vi "Enregistrer_fichier_profil EPC3000.vi"(2 "error in (no error) 2":errorcluster caption="entrée d'erreur (pas d'erreur)", 3 "Config + programmes":T1 {"Prog 10 en sortie"."?" format="%#.1f"; "Prog 9 en sortie"."?" format="%#.1f"; "Prog 8 en sortie"."?" format="%#.1f"; "Prog 7 en sortie"."?" format="%#.1f"; "Prog 6 en sortie"."?" format="%#.1f"; "Prog 5 en sortie"."?" format="%#.1f"; "config"."value" format="%#.1f"; "Prog 1 en sortie"."?" format="%#.1f"; "Prog 2 en sortie"."?" format="%#.1f"; "Prog 3 en sortie"."?" format="%#.1f"; "Prog 4 en sortie"."?" format="%#.1f"}, 4 "Chemin du fichier profil":path caption="chemin du fichier de configuration") -> (0 "error out 2":errorcluster caption="entrée d'erreur (pas d'erreur)", 1 "Chemin de fichier en sortie":path caption="Chemin du fichier en sortie")   [LabVIEW 2022 SP3]
uses:
  <vilib>/Utility/config.llb/Write Key (Double).vi
  <vilib>/Utility/config.llb/NI_LVConfig.lvlib
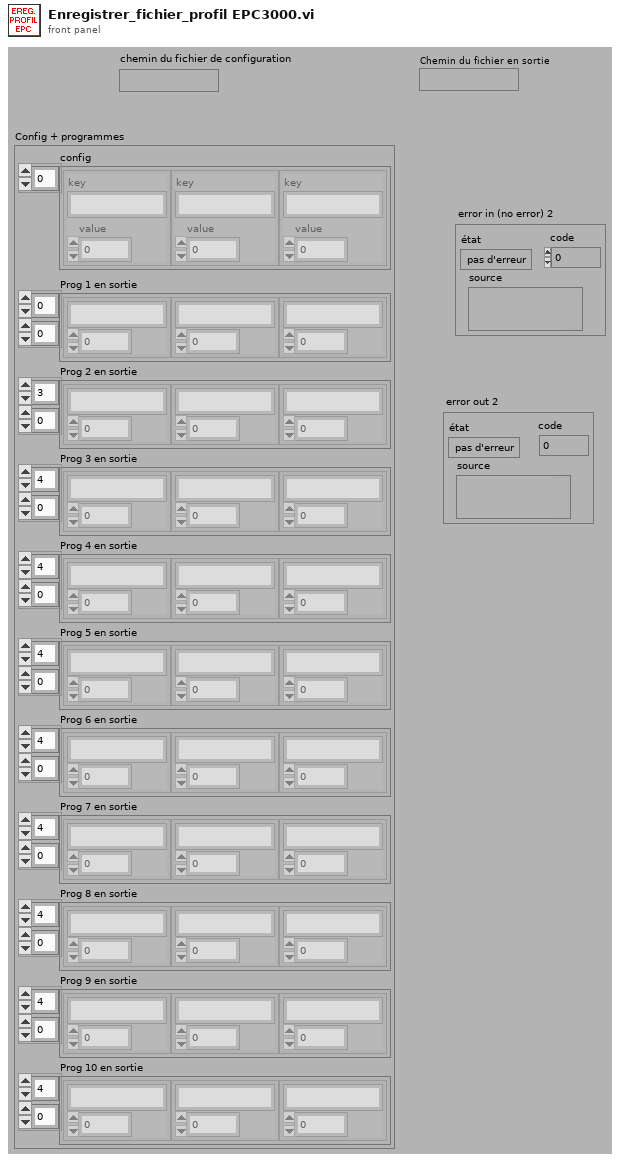
[diagram p1: front panel]
types:
  T1 = cluster{"config":cluster{"key":string, "value":dbl}[], "Prog 1 en sortie":cluster{string, dbl}[][], "Prog 2 en sortie":cluster{string, dbl}[][], "Prog 3 en sortie":cluster{string, dbl}[][], "Prog 4 en sortie":cluster{string, dbl}[][], "Prog 5 en sortie":cluster{string, dbl}[][], "Prog 6 en sortie":cluster{string, dbl}[][], "Prog 7 en sortie":cluster{string, dbl}[][], "Prog 8 en sortie":cluster{string, dbl}[][], "Prog 9 en sortie":cluster{string, dbl}[][], "Prog 10 en sortie":cluster{string, dbl}[][]}
  T2 = typedef "NI_LVConfig.lvlib/Config Data RefNum.ctl" = refnum<k1>
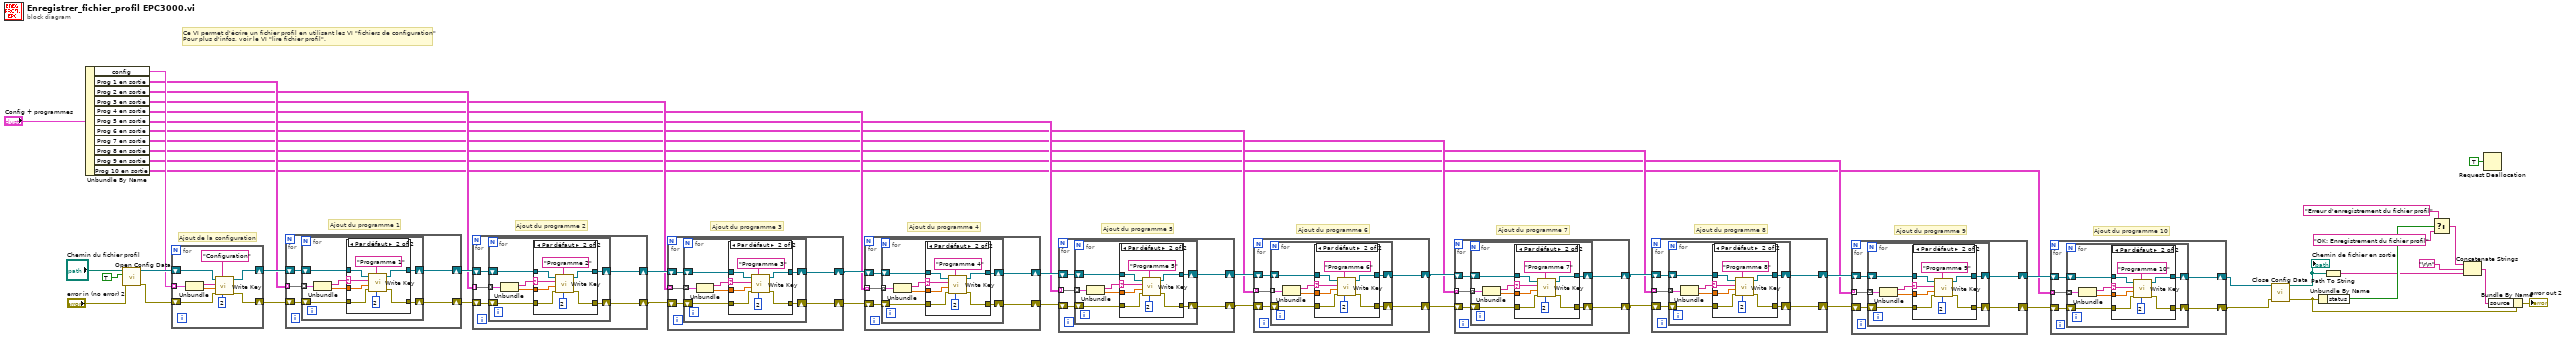
[diagram p0: block diagram]
diagram:
  # "Ajout du programme 10"
  # "Ajout du programme 9"
  # "Ajout du programme 8"
  # "Ajout du programme 7"
  # "Ajout du programme 6"
  # "Ajout du programme 5"
  # "Ajout du programme 4"
  # "Ajout du programme 3"
  # "Ajout du programme 2"
  # "Ce VI permet d'écrire un fichier profil en utilisant les VI \"fichiers de configuration\"\nPour plus d'infos, voir le VI \"lire fichier profil\"."
  # "Ajout du programme 1"
  # "Ajout de la configuration"
  n1 = Unbundle By Name("Config + programmes") -> ("config"=w31:cluster{"key":string, "value":dbl}[], "Prog 1 en sortie"=w30:cluster{string, dbl}[][], "Prog 2 en sortie"=w27:cluster{string, dbl}[][], "Prog 3 en sortie"=w24:cluster{string, dbl}[][], "Prog 4 en sortie"=w21:cluster{string, dbl}[][], "Prog 5 en sortie"=w18:cluster{string, dbl}[][], "Prog 6 en sortie"=w15:cluster{string, dbl}[][], "Prog 7 en sortie"=w12:cluster{string, dbl}[][], "Prog 8 en sortie"=w9:cluster{string, dbl}[][], "Prog 9 en sortie"=w6:cluster{string, dbl}[][], "Prog 10 en sortie"=w3:cluster{string, dbl}[][])
  n2 = call <vilib>:"Open Config Data.vi"("error in (no error)"="error in (no error) 2", "create file if necessary (T)"=TRUE ("create file if necessary? (T)"), "configuration file path"="Chemin du fichier profil") -> ("error out"=w45:errorcluster, "refnum"=w46:T2)  [unwired: 6 in, 1 out]
  n3 = for {
    tunnel: w31 -> [w59] mode=indexing
    shift-right: [w54] -> w47
    shift-left: w45 -> [w55]
    shift-right: [w53] -> w48
    shift-left: w46 -> [w52]
    n4 = Unbundle(w59) -> ("key"=w57:string, "value"=w56:dbl)
    n5 = call-poly <vilib>:"Write Key.vi"("precision (6)"=i16 2, "section"="Configuration", "error in (no error)"=w55, "value"=w56, "key"=w57, "refnum"=w52) -> ("error out"=w54:errorcluster, "refnum out"=w53:T2)  [unwired: 3 in, 1 out]
  }
  n6 = for {
    tunnel: w30 -> [w62] mode=indexing
    shift-right: [w60] -> w29
    shift-left: w47 -> [w64]
    shift-right: [w61] -> w28
    shift-left: w48 -> [w63]
    n7 = for {
      tunnel: w62 -> [w67] mode=indexing
      shift-right: [w69] -> w61
      shift-left: w63 -> [w68]
      shift-right: [w70] -> w60
      shift-left: w64 -> [w71]
      n8 = Unbundle(w67) -> (w66:string, w65:dbl)
      n9 = case shown="Par défaut" w66 {
        selector: w66 -> [_ w75]
        tunnel: w71 -> [w72 w80]
        tunnel: [w72 w79] -> w70
        tunnel: [w73 w78] -> w69
        tunnel: w68 -> [w73 w77]
        tunnel: w65 -> [_ w76]
        frame "" {
        }
        frame Default {
          n10 = call-poly <vilib>:"Write Key.vi"("precision (6)"=i16 2, "section"="Programme 1", "error in (no error)"=w80, "value"=w76, "key"=w75, "refnum"=w77) -> ("error out"=w79:errorcluster, "refnum out"=w78:T2)  [unwired: 3 in, 1 out]
        }
      }
    }
  }
  n11 = for {
    tunnel: w27 -> [w84] mode=indexing
    shift-right: [w82] -> w25
    shift-left: w29 -> [w86]
    shift-right: [w83] -> w26
    shift-left: w28 -> [w85]
    n12 = for {
      tunnel: w84 -> [w89] mode=indexing
      shift-right: [w91] -> w83
      shift-left: w85 -> [w90]
      shift-right: [w92] -> w82
      shift-left: w86 -> [w93]
      n13 = Unbundle(w89) -> (w88:string, w87:dbl)
      n14 = case shown="Par défaut" w88 {
        selector: w88 -> [_ w97]
        tunnel: w93 -> [w94 w102]
        tunnel: [w94 w101] -> w92
        tunnel: [w95 w100] -> w91
        tunnel: w90 -> [w95 w99]
        tunnel: w87 -> [_ w98]
        frame "" {
        }
        frame Default {
          n15 = call-poly <vilib>:"Write Key.vi"("precision (6)"=i16 2, "section"="Programme 2", "error in (no error)"=w102, "value"=w98, "key"=w97, "refnum"=w99) -> ("error out"=w101:errorcluster, "refnum out"=w100:T2)  [unwired: 3 in, 1 out]
        }
      }
    }
  }
  n16 = for {
    tunnel: w24 -> [w106] mode=indexing
    shift-right: [w104] -> w22
    shift-left: w25 -> [w108]
    shift-right: [w105] -> w23
    shift-left: w26 -> [w107]
    n17 = for {
      tunnel: w106 -> [w111] mode=indexing
      shift-right: [w113] -> w105
      shift-left: w107 -> [w112]
      shift-right: [w114] -> w104
      shift-left: w108 -> [w115]
      n18 = Unbundle(w111) -> (w110:string, w109:dbl)
      n19 = case shown="Par défaut" w110 {
        selector: w110 -> [_ w119]
        tunnel: w115 -> [w116 w124]
        tunnel: [w116 w123] -> w114
        tunnel: [w117 w122] -> w113
        tunnel: w112 -> [w117 w121]
        tunnel: w109 -> [_ w120]
        frame "" {
        }
        frame Default {
          n20 = call-poly <vilib>:"Write Key.vi"("precision (6)"=i16 2, "section"="Programme 3", "error in (no error)"=w124, "value"=w120, "key"=w119, "refnum"=w121) -> ("error out"=w123:errorcluster, "refnum out"=w122:T2)  [unwired: 3 in, 1 out]
        }
      }
    }
  }
  n21 = for {
    tunnel: w21 -> [w128] mode=indexing
    shift-right: [w126] -> w19
    shift-left: w22 -> [w130]
    shift-right: [w127] -> w20
    shift-left: w23 -> [w129]
    n22 = for {
      tunnel: w128 -> [w133] mode=indexing
      shift-right: [w135] -> w127
      shift-left: w129 -> [w134]
      shift-right: [w136] -> w126
      shift-left: w130 -> [w137]
      n23 = Unbundle(w133) -> (w132:string, w131:dbl)
      n24 = case shown="Par défaut" w132 {
        selector: w132 -> [_ w141]
        tunnel: w137 -> [w138 w146]
        tunnel: [w138 w145] -> w136
        tunnel: [w139 w144] -> w135
        tunnel: w134 -> [w139 w143]
        tunnel: w131 -> [_ w142]
        frame "" {
        }
        frame Default {
          n25 = call-poly <vilib>:"Write Key.vi"("precision (6)"=i16 2, "section"="Programme 4", "error in (no error)"=w146, "value"=w142, "key"=w141, "refnum"=w143) -> ("error out"=w145:errorcluster, "refnum out"=w144:T2)  [unwired: 3 in, 1 out]
        }
      }
    }
  }
  n26 = for {
    tunnel: w18 -> [w150] mode=indexing
    shift-right: [w148] -> w16
    shift-left: w19 -> [w152]
    shift-right: [w149] -> w17
    shift-left: w20 -> [w151]
    n27 = for {
      tunnel: w150 -> [w155] mode=indexing
      shift-right: [w157] -> w149
      shift-left: w151 -> [w156]
      shift-right: [w158] -> w148
      shift-left: w152 -> [w159]
      n28 = Unbundle(w155) -> (w154:string, w153:dbl)
      n29 = case shown="Par défaut" w154 {
        selector: w154 -> [_ w163]
        tunnel: w159 -> [w160 w168]
        tunnel: [w160 w167] -> w158
        tunnel: [w161 w166] -> w157
        tunnel: w156 -> [w161 w165]
        tunnel: w153 -> [_ w164]
        frame "" {
        }
        frame Default {
          n30 = call-poly <vilib>:"Write Key.vi"("precision (6)"=i16 2, "section"="Programme 5", "error in (no error)"=w168, "value"=w164, "key"=w163, "refnum"=w165) -> ("error out"=w167:errorcluster, "refnum out"=w166:T2)  [unwired: 3 in, 1 out]
        }
      }
    }
  }
  n31 = for {
    tunnel: w15 -> [w172] mode=indexing
    shift-right: [w170] -> w13
    shift-left: w16 -> [w174]
    shift-right: [w171] -> w14
    shift-left: w17 -> [w173]
    n32 = for {
      tunnel: w172 -> [w177] mode=indexing
      shift-right: [w179] -> w171
      shift-left: w173 -> [w178]
      shift-right: [w180] -> w170
      shift-left: w174 -> [w181]
      n33 = Unbundle(w177) -> (w176:string, w175:dbl)
      n34 = case shown="Par défaut" w176 {
        selector: w176 -> [_ w185]
        tunnel: w181 -> [w182 w190]
        tunnel: [w182 w189] -> w180
        tunnel: [w183 w188] -> w179
        tunnel: w178 -> [w183 w187]
        tunnel: w175 -> [_ w186]
        frame "" {
        }
        frame Default {
          n35 = call-poly <vilib>:"Write Key.vi"("precision (6)"=i16 2, "section"="Programme 6", "error in (no error)"=w190, "value"=w186, "key"=w185, "refnum"=w187) -> ("error out"=w189:errorcluster, "refnum out"=w188:T2)  [unwired: 3 in, 1 out]
        }
      }
    }
  }
  n36 = for {
    tunnel: w12 -> [w194] mode=indexing
    shift-right: [w192] -> w10
    shift-left: w13 -> [w196]
    shift-right: [w193] -> w11
    shift-left: w14 -> [w195]
    n37 = for {
      tunnel: w194 -> [w199] mode=indexing
      shift-right: [w201] -> w193
      shift-left: w195 -> [w200]
      shift-right: [w202] -> w192
      shift-left: w196 -> [w203]
      n38 = Unbundle(w199) -> (w198:string, w197:dbl)
      n39 = case shown="Par défaut" w198 {
        selector: w198 -> [_ w207]
        tunnel: w203 -> [w204 w212]
        tunnel: [w204 w211] -> w202
        tunnel: [w205 w210] -> w201
        tunnel: w200 -> [w205 w209]
        tunnel: w197 -> [_ w208]
        frame "" {
        }
        frame Default {
          n40 = call-poly <vilib>:"Write Key.vi"("precision (6)"=i16 2, "section"="Programme 7", "error in (no error)"=w212, "value"=w208, "key"=w207, "refnum"=w209) -> ("error out"=w211:errorcluster, "refnum out"=w210:T2)  [unwired: 3 in, 1 out]
        }
      }
    }
  }
  n41 = for {
    tunnel: w9 -> [w216] mode=indexing
    shift-right: [w214] -> w7
    shift-left: w10 -> [w218]
    shift-right: [w215] -> w8
    shift-left: w11 -> [w217]
    n42 = for {
      tunnel: w216 -> [w221] mode=indexing
      shift-right: [w223] -> w215
      shift-left: w217 -> [w222]
      shift-right: [w224] -> w214
      shift-left: w218 -> [w225]
      n43 = Unbundle(w221) -> (w220:string, w219:dbl)
      n44 = case shown="Par défaut" w220 {
        selector: w220 -> [_ w229]
        tunnel: w225 -> [w226 w234]
        tunnel: [w226 w233] -> w224
        tunnel: [w227 w232] -> w223
        tunnel: w222 -> [w227 w231]
        tunnel: w219 -> [_ w230]
        frame "" {
        }
        frame Default {
          n45 = call-poly <vilib>:"Write Key.vi"("precision (6)"=i16 2, "section"="Programme 8", "error in (no error)"=w234, "value"=w230, "key"=w229, "refnum"=w231) -> ("error out"=w233:errorcluster, "refnum out"=w232:T2)  [unwired: 3 in, 1 out]
        }
      }
    }
  }
  n46 = for {
    tunnel: w6 -> [w238] mode=indexing
    shift-right: [w236] -> w4
    shift-left: w7 -> [w240]
    shift-right: [w237] -> w5
    shift-left: w8 -> [w239]
    n47 = for {
      tunnel: w238 -> [w243] mode=indexing
      shift-right: [w245] -> w237
      shift-left: w239 -> [w244]
      shift-right: [w246] -> w236
      shift-left: w240 -> [w247]
      n48 = Unbundle(w243) -> (w242:string, w241:dbl)
      n49 = case shown="Par défaut" w242 {
        selector: w242 -> [_ w251]
        tunnel: w247 -> [w248 w256]
        tunnel: [w248 w255] -> w246
        tunnel: [w249 w254] -> w245
        tunnel: w244 -> [w249 w253]
        tunnel: w241 -> [_ w252]
        frame "" {
        }
        frame Default {
          n50 = call-poly <vilib>:"Write Key.vi"("precision (6)"=i16 2, "section"="Programme 9", "error in (no error)"=w256, "value"=w252, "key"=w251, "refnum"=w253) -> ("error out"=w255:errorcluster, "refnum out"=w254:T2)  [unwired: 3 in, 1 out]
        }
      }
    }
  }
  n51 = for {
    tunnel: w3 -> [w260] mode=indexing
    shift-right: [w258] -> w1
    shift-left: w4 -> [w262]
    shift-right: [w259] -> w2
    shift-left: w5 -> [w261]
    n52 = for {
      tunnel: w260 -> [w265] mode=indexing
      shift-right: [w267] -> w259
      shift-left: w261 -> [w266]
      shift-right: [w268] -> w258
      shift-left: w262 -> [w269]
      n53 = Unbundle(w265) -> (w264:string, w263:dbl)
      n54 = case shown="Par défaut" w264 {
        selector: w264 -> [_ w273]
        tunnel: w269 -> [w270 w278]
        tunnel: [w270 w277] -> w268
        tunnel: [w271 w276] -> w267
        tunnel: w266 -> [w271 w275]
        tunnel: w263 -> [_ w274]
        frame "" {
        }
        frame Default {
          n55 = call-poly <vilib>:"Write Key.vi"("precision (6)"=i16 2, "section"="Programme 10", "error in (no error)"=w278, "value"=w274, "key"=w273, "refnum"=w275) -> ("error out"=w277:errorcluster, "refnum out"=w276:T2)  [unwired: 3 in, 1 out]
        }
      }
    }
  }
  n56 = call <vilib>:"Close Config Data.vi"("error in (no error)"=w1, "refnum"=w2) -> ("error out"=w36:errorcluster, "file path"=w44:path)  [unwired: 8 in]
  "Chemin de fichier en sortie" <- w44
  n57 = Unbundle By Name(w36) -> ("status"=w42:bool)
  n58 = Path To String(path=w44) -> (string=w37:string)
  n59 = Select(t="Erreur d'enregistrement du fichier profil", s=w42, f="OK: Enregistrement du fichier profil") -> (s? t:f=w38:string)
  n60 = Concatenate Strings(w38, "\r\n", w37) -> (w35:string)
  n61 = Request Deallocation(TRUE ("flag")) -> ()
  n62 = Bundle By Name(cluster=w36, "source"=w35) -> (→"error out 2":errorcluster)
